vi "Set Multi-Line Package Attribute Value.vi"(0 "package attributes string in":string, 5 "package attribute name":string, 7 "synopsis":string, 9 "description":string, 11 "error in (no error)":errorcluster, 12 "add nonexisting attribute to string (T)":bool=TRUE) -> (4 "package attributes string out":string, 6 "new attribute added to string?":bool, 8 "attribute found?":bool, 15 "error out":errorcluster)   [LabVIEW 2014, in "NIPM_API.lvlib"]
doc: "Sets the value for an attribute in a package attribute string.\n\nINPUT(s)\n<B>Package attributes string in</B>: This is the initial string containing the package attributes. For example, this string could come from reading the contents of an unpacked package's control file.\n\n<B>Package attribute name</B>: This is the name of the attribute whose value you want to change.\n\n<B>Package attribute value</B>: This is the value you want to set the attribute to.\n\n<B>Add nonexisting attribute to string</B>: If this VI does not find the \"package attribute name\" in the \"package attributes string in\" string, this input determines whether this VI will add the \"package attribute name\" and \"package attribute value\" to the \"package attribute string\".\nNote: If this input is TRUE, but the \"package attribute value\" is a default value (\"\"), then this VI will not add a new attribute to the string.\n\nOUTPUT(s)\n<B>Package attributes string out</B>: Outputs the modified package attributes string that contains the new value(s)\n\n<B>New attribute added to string?</B>: This output will be TRUE if a new attribute (did not exist in the incoming \"package attributes string in\" string) was added to the package attributes string.\n\n<B>Attribute found?</B>: This output will be TRUE if the \"package attribute name\" was found in the incoming \"package attributes string in\" string."
uses:
  NIPM_API.lvlib
  <vilib>/Utility/error.llb/whitespace.ctl
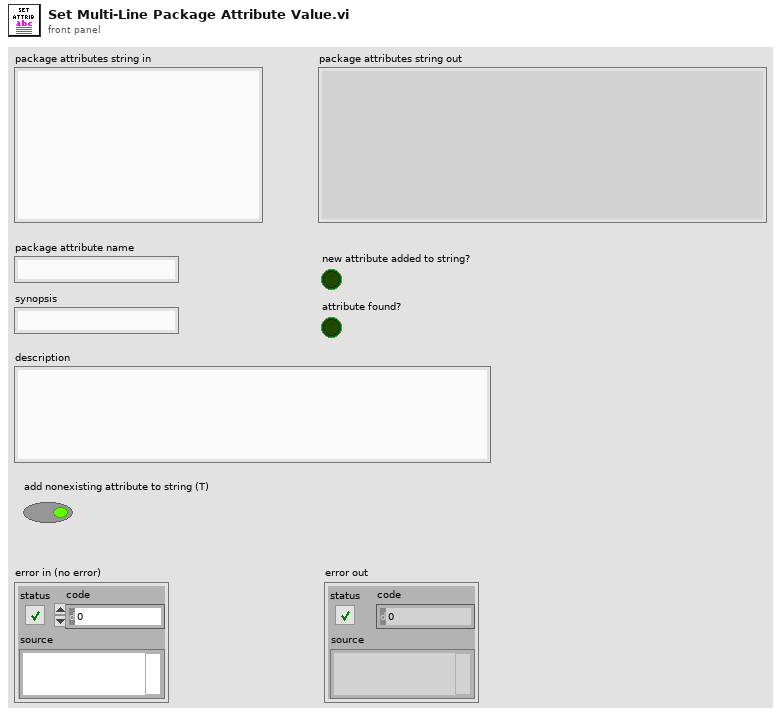
[diagram p1: front panel]
types:
  T1 = typedef "whitespace.ctl" = u16
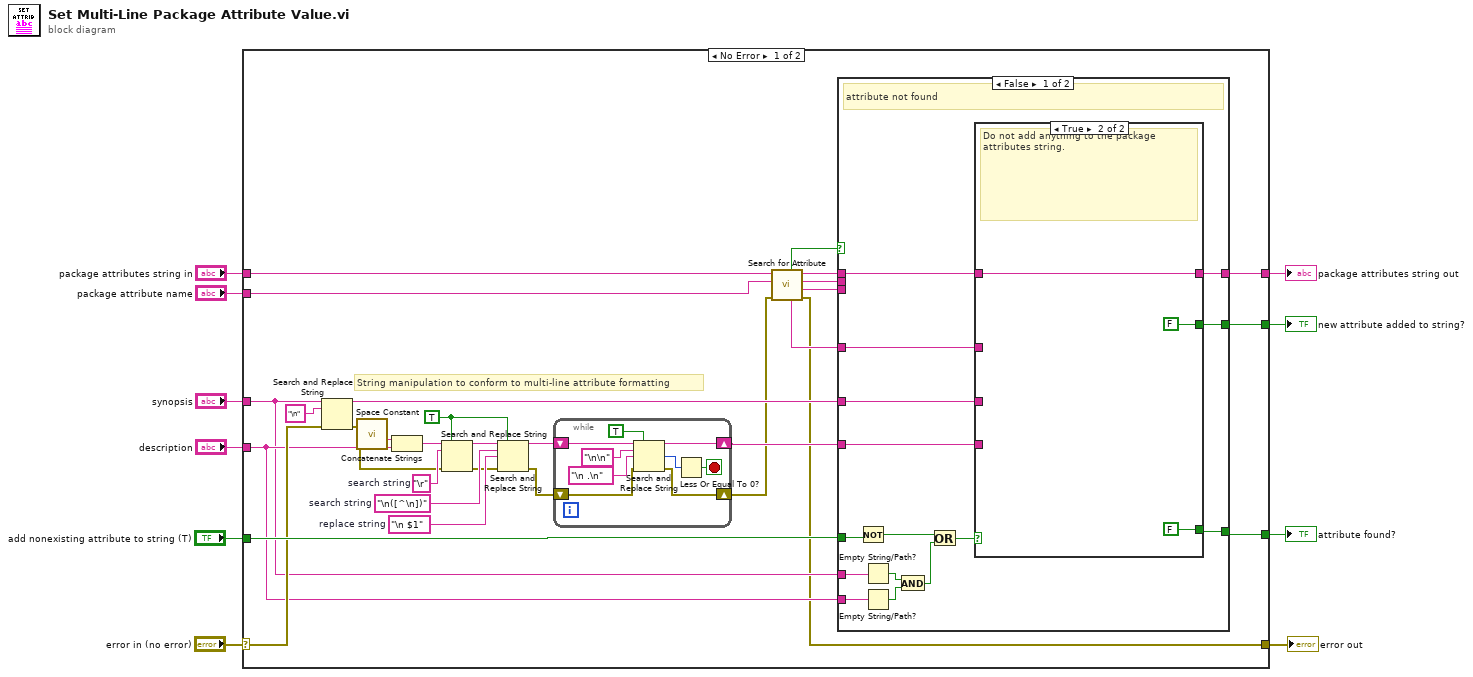
[diagram p0: block diagram]
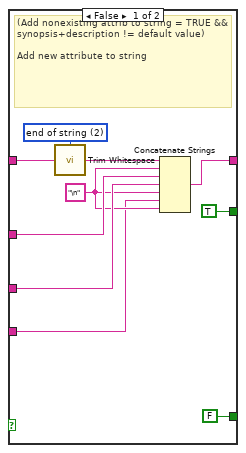
[diagram p2: hidden frame]
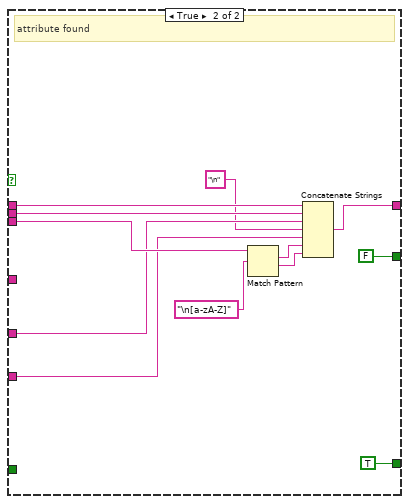
[diagram p3: hidden frame]
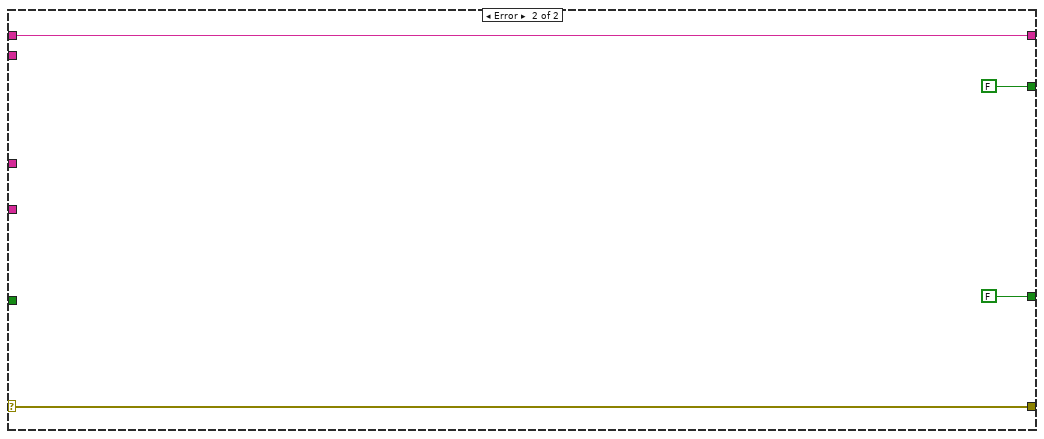
[diagram p4: hidden frame]
diagram:
  n1 = case shown="No Error" "error in (no error)" {
    selector: "error in (no error)" -> [w34 w93]
    tunnel: [w40 w90] -> w10
    tunnel: "package attribute name" -> [w19 _]
    tunnel: "package attributes string in" -> [w25 w90]
    tunnel: [w17 w93] -> w6
    tunnel: "description" -> [w27 _]
    tunnel: [w39 FALSE] -> w4
    tunnel: "add nonexisting attribute to string (T)" -> [w38 _]
    tunnel: [w37 FALSE] -> w2
    tunnel: "synopsis" -> [w26 _]
    frame No Error {
      w14 = "\r"  # search string
      w13 = TRUE ("replace all? (F)")
      w29 = "\n $1"  # replace string
      w30 = "\n([^\n])"  # search string
      # "String manipulation to conform to multi-line attribute formatting"
      n2 = Search and Replace String(input string=w26, search string="\n" ("regular expression"), error in=w34) -> (result string=w35:string, error out=w12:errorcluster)  [unwired: 5 in, 2 out]
      n3 = call <vilib>:"Space Constant.vi"() -> ("String"=w33:string)
      n4 = Concatenate Strings(w33, w27) -> (w15:string)
      n5 = Search and Replace String(replace all?=w13, input string=w15, search string=w14, error in=w12) -> (result string=w16:string, error out=w11:errorcluster)  [unwired: 4 in, 2 out]
      n6 = Search and Replace String(replace all?=w13, input string=w16, search string=w30, replace string=w29, error in=w11) -> (result string=w31:string, error out=w28:errorcluster)  [unwired: 3 in, 2 out]
      n7 = while {
        shift-right: [w46] -> w32
        shift-left: w31 -> [w49]
        shift-right: [w42] -> w18
        shift-left: w28 -> [w43]
        stop <- w44 stop-if-true
        n8 = Search and Replace String(replace all?=TRUE ("replace all? (F)"), input string=w49, search string="\n\n" ("regular expression"), replace string="\n .\n" ("regular expression"), error in=w43) -> (result string=w46:string, number of replacements=w45:i32, error out=w42:errorcluster)  [unwired: 3 in, 1 out]
        n9 = Less Or Equal To 0?(x=w45) -> (x <= 0?=w44:bool)
      }
      n10 = call "Search for Attribute.vi"("error in (no error)"=w18, "package attribute name"=w19, "package attributes CLI string in"=w25) -> ("error out"=w17:errorcluster, "string after attribute"=w22:string, "string matching attribute"=w23:string, "string before attribute"=w24:string, "package attribute string"=w20:string, "attribute found?"=w21:bool)  [unwired: 3 in]
      n11 = case shown="False" w21 {
        tunnel: w24 -> [w64 w89]
        tunnel: w23 -> [_ w88]
        tunnel: w32 -> [w60 w80]
        tunnel: w22 -> [_ w87]
        tunnel: [w62 w86] -> w40
        tunnel: [w63 FALSE] -> w39
        tunnel: w20 -> [w61 _]
        tunnel: w38 -> [w57 _]
        tunnel: [w59 TRUE] -> w37
        tunnel: w35 -> [w58 w81]
        tunnel: w27 -> [w53 _]
        tunnel: w26 -> [w54 _]
        frame False {
          # "attribute not found"
          n12 = Not(x=w57) -> (.not. x?=w55:bool)
          n13 = Empty String/Path?(string/path=w54) -> (empty?=w52:bool)
          n14 = Empty String/Path?(string/path=w53) -> (empty?=w51:bool)
          n15 = And(x=w52, y=w51) -> (x .and. y?=w50:bool)
          n16 = Or(x=w55, y=w50) -> (x .or. y?=w56:bool)
          n17 = case shown="True" w56 {
            tunnel: w64 -> [w74 w77]
            tunnel: [TRUE FALSE] -> w63
            tunnel: [w72 w77] -> w62
            tunnel: w61 -> [w71 _]
            tunnel: w60 -> [w65 _]
            tunnel: [FALSE FALSE] -> w59
            tunnel: w58 -> [w67 _]
            frame False {
              w66 = "\n"
              w69 = T1 2 items=["both", "start of string", "end of string"] ("location (both)")
              # "(Add nonexisting attrib to string = TRUE && synopsis+description != default value)\n\nAdd new attribute to string"
              n18 = call <vilib>:"Trim Whitespace.vi"("string"=w74, "location (both)"=w69) -> ("trimmed string"=w70:string)
              n19 = Concatenate Strings(w70, w66, w71, w67, w66, w65, w66) -> (w72:string)
            }
            frame True {
              # "Do not add anything to the package attributes string."
            }
          }
        }
        frame True {
          # "attribute found"
          n20 = Match Pattern(string=w87, regular expression="\n[a-zA-Z]" ("Package Attribute Name")) -> (match substring=w84:string, after substring=w83:string)  [unwired: 1 in, 2 out]
          n21 = Concatenate Strings(w89, w88, w81, "\n" ("regular expression"), w80, w84, w83) -> (w86:string)
        }
      }
    }
    frame Error {
    }
  }
  "package attributes string out" <- w10
  "error out" <- w6
  "new attribute added to string?" <- w4
  "attribute found?" <- w2
